vi "General Glob.vi"() -> ()   [LabVIEW 2025]
panel:
  out "RFM (lb/h)":dbl
  out "Ref Capacity (BTU / h)":dbl
  out "pt (psi)":dbl format="%0.2f"
  out "off coil WBT (F)":dbl format="%0.2f"
  out "off coil DBT (F)":dbl format="%0.2f"
  out "on coil WBT (F)":dbl format="%0.2f"
  out "on coil DBT (F)":dbl format="%0.2f"
  out "Noz DP":dbl format="%0.2f"
  out "Noz SP":dbl format="%0.2f"
  out "Latent Cap Air":dbl format="%0.2f"
  out "Sensible Cap Air":dbl format="%0.2f"
  out "Specific Vol Supply":dbl format="%0.2f"
  out "Humidity Ratio Supply":dbl format="%0.2f"
  out "FCU WPD":dbl format="%0.2f"
  out "FCU EWT":dbl format="%0.2f"
  out "FCU LWT":dbl format="%0.2f"
  out "FCU WFR":dbl format="%0.2f"
  out "Water Capacity":dbl format="%0.2f"
  out "HB":dbl format="%0.2f"
  out "ACFM":dbl format="%0.2f"
  out "SCFM":dbl format="%0.2f"
  out "ESP":dbl format="%0.2f"
  out "COP":dbl format="%0.2f"
  out "Air Capacity":dbl format="%0.2f"
  out "ID Entering WB":dbl format="%0.2f"
  out "ID Entering DB":dbl format="%0.2f"
  out "ID Leaving DB":dbl format="%0.2f"
  out "ID Leaving WB":dbl format="%0.2f"
  out "Delta DBT":dbl format="%0.2f"
  out "Delta WBT":dbl format="%0.2f"
  out "Condensing Temp":dbl
  out "Evaporating Temp":dbl
  in  "Liquid  Temp":u16(ring) items=["ID_TC 01", "ID_TC 02", "ID_TC 03", "ID_TC 04", "ID_TC 05", "ID_TC 06", "ID_TC 07", "ID_TC 08", "ID_TC 09", "ID_TC 10", "ID_TC 11", "ID_TC 12", "ID_TC 13", "ID_TC 14", "ID_TC 15", "ID_TC 16"]
  in  "Discharge Temp":u16(ring) items=["OD_TC 01", "OD_TC 02", "OD_TC 03", "OD_TC 04", "OD_TC 05", "OD_TC 06", "OD_TC 07", "OD_TC 08", "OD_TC 09", "OD_TC 10", "OD_TC 11", "OD_TC 12", "OD_TC 13", "OD_TC 14", "OD_TC 15", "OD_TC 16"]
  in  "Suction Temp":u16(ring) items=["OD_TC 01", "OD_TC 02", "OD_TC 03", "OD_TC 04", "OD_TC 05", "OD_TC 06", "OD_TC 07", "OD_TC 08", "OD_TC 09", "OD_TC 10", "OD_TC 11", "OD_TC 12", "OD_TC 13", "OD_TC 14", "OD_TC 15", "OD_TC 16"]
  out "Super Heat":dbl
  out "Sub Cool":dbl
  out "Initial weight (ID Cooling Coil Cond)":dbl
  out "Initial weight (UUT Cond)":dbl
  out "initial Time at\n start Record":timestamp=timestamp(3628411169.8998337 s since 1904-01-01) format="%<%I:%M:%S %p\n%d/%m/%Y>T"
  in  "Configuration Data":T1={"Refrigerant"=enum."R410a", "Unit Model"="", "Job Number"="", "Reported by"="", "Testing Period (min)"=30.0, "Sampling Freq (Sec)"=5.0}
  out "STOP Program":bool
  out "ID Total Cooling Capacity":dbl
  out "OD Total Cooling Capacity":dbl
  out "Finished Inputs":bool
  out "Stop Test/PMs":bool
  out "Specific Enthalpy Vapor":dbl[](array[numeric])
  in  "OD Heat leak Partition":dbl
  in  "ODHeat leak Walls":dbl
  out "Time Stamp":string
  out "Heat Leakag /Walls ID":dbl
  out "Heat Leakag /Partition ID":dbl
  out "hw3 Return Condensed OD":dbl
  out "hw2 Return Condensed ID":dbl
  out "hw1 Supply Staem":dbl
  in  "Section 1: Testing Laboratory":T2
  in  "Section 2: Product Specification":T3
  out "Readings Counter  lng":dbl
  out "Test Record":bool
  out "Readings Counter sml":dbl
  out "Total Number of Readings":dbl
  out "Fetch data":dbl
  out "System Status":string
  out "Specific Enthalpy Liquid":dbl[](array[numeric])
  out "Temperatures fo Enthalpy":dbl[](array[numeric])
  # "Indoor Capacity"
  # "Input Parameters"
  # "gram"
  # "W"
  # "gram"
  # "W"
  # "W"
  # "Outdoor Capacity"
  # "Water side Capacity"
  # "Air side Capacity"
  # "DBT"
  # "WBT"
  # "Return"
  # "C"
  # "C"
  # "Supply"
  # "C"
  # "C"
  # "C"
  # "Diff"
  # "gpm"
  # "W"
  # "Pa"
  # "W/W"
  # "W"
  # "%"
  # "W"
  # "Pa"
  # "Refrigerant Data"
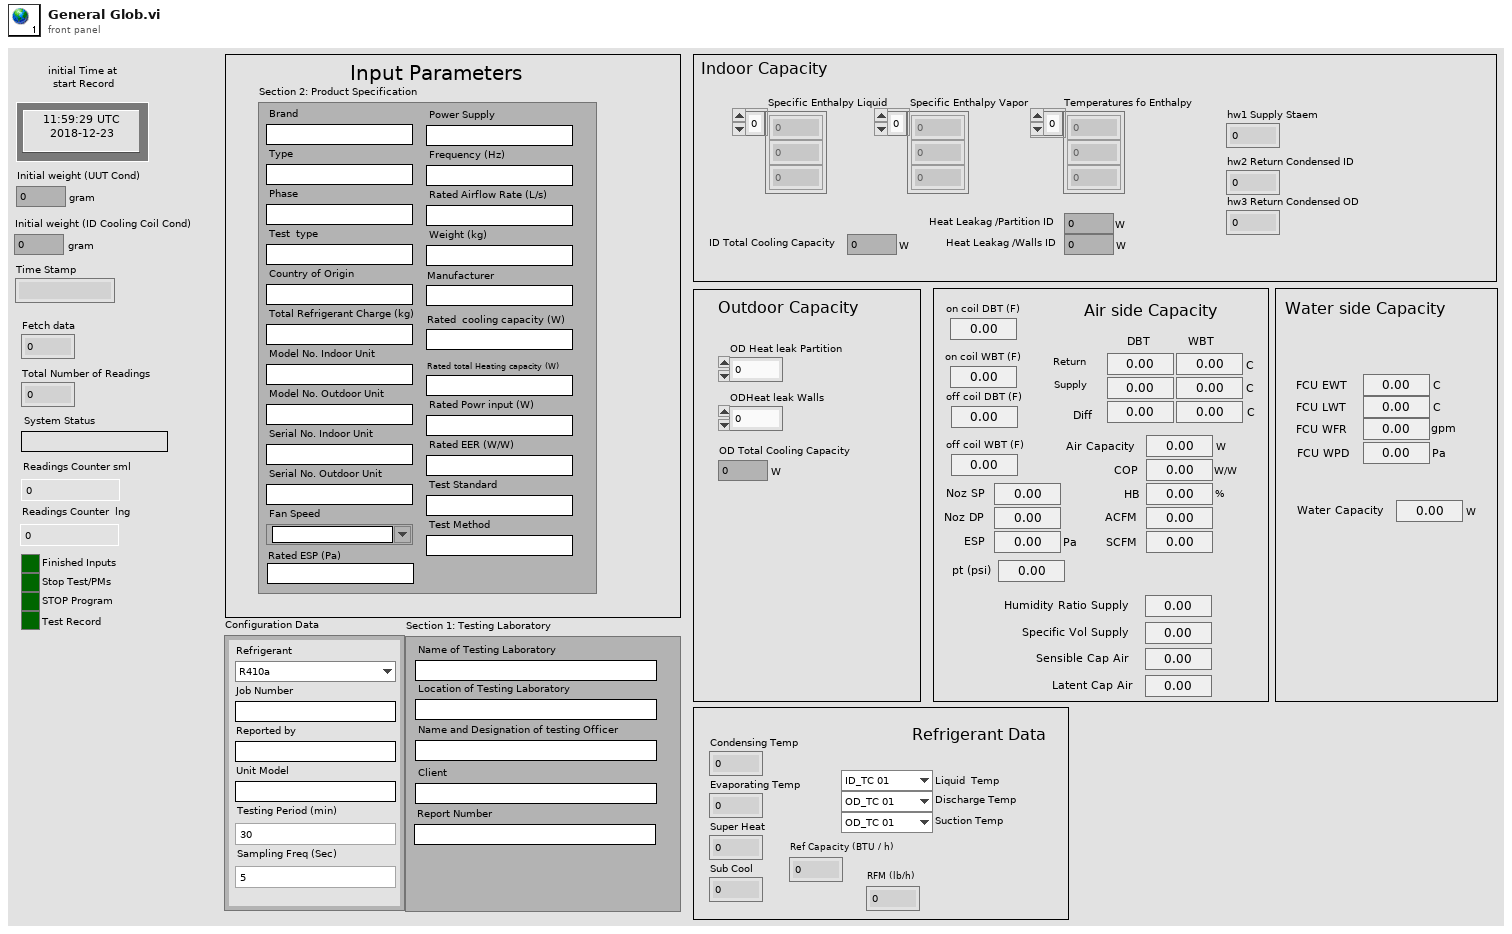
[diagram p1: front panel]
types:
  T1 = cluster{"Refrigerant":enum16{"R407c", "R410a", "R134a", "R22", ""}, "Unit Model":string, "Job Number":string, "Reported by":string, "Testing Period (min)":dbl, "Sampling Freq (Sec)":dbl}
  T2 = cluster{"Name of Testing Laboratory":string, "Location of Testing Laboratory":string, "Name and Designation of testing Officer":string, "Client":string, "Report Number":string}
  T3 = cluster{"Brand":string, "Type":string, "Phase":string, "Test  type":string, "Country of Origin":string, "Total Refrigerant Charge (kg)":string, "Power Supply":string, "Frequency (Hz)":string, "Rated Airflow Rate (L/s)":string, "Manufacturer":string, "Weight (kg)":string, "Rated  cooling capacity (W)":string, "Rated Powr input (W)":string, "Test Standard":string, "Test Method":string, "Model No. Indoor Unit":string, "Model No. Outdoor Unit":string, "Serial No. Indoor Unit":string, "Serial No. Outdoor Unit":string, "Rated EER (W/W)":string, "Rated total Heating capacity (W)":string, "Fan Speed ":string, "Rated ESP (Pa)":string}
diagram:
